vi "Read Sequence File.vi"(8 "error in":errorcluster, 11 "path":path) -> (0 "error out":errorcluster, 2 "rig config path":path, 3 "Sequence File":T1)   [LabVIEW 2026]
doc: "Reads a sequence JSON file as text and parses it with Parse Sequence JSON.vi into a Sequence File cluster; the rig config path is the sequence file folder joined with rig_config. An empty path returns error 7; a missing file, a JSON error or an empty steps array (error 5001) is passed out. AF-free."
uses:
  Typedefs/Condition.ctl
  Typedefs/Channel Value.ctl
  Typedefs/Step Config.ctl
  Typedefs/Sequence File.ctl
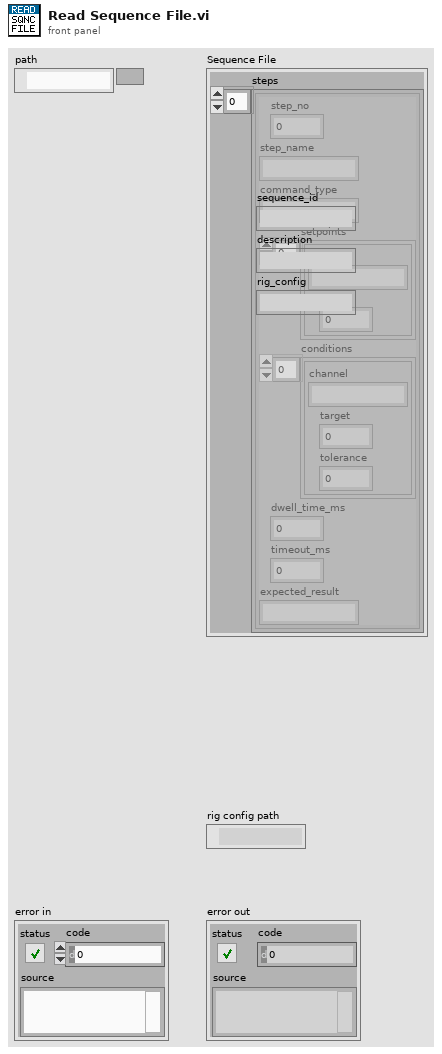
[diagram p1: front panel]
types:
  T1 = typedef "Sequence File.ctl" = cluster{"sequence_id":string, "description":string, "rig_config":string, "steps":T2[]}
  T2 = typedef "Step Config.ctl" = cluster{"step_no":i32, "step_name":string, "command_type":string, "setpoints":T3[], "conditions":T4[], "dwell_time_ms":i32, "timeout_ms":i32, "expected_result":string}
  T3 = typedef "Channel Value.ctl" = cluster{"channel":string, "value":dbl}
  T4 = typedef "Condition.ctl" = cluster{"channel":string, "target":dbl, "tolerance":dbl}
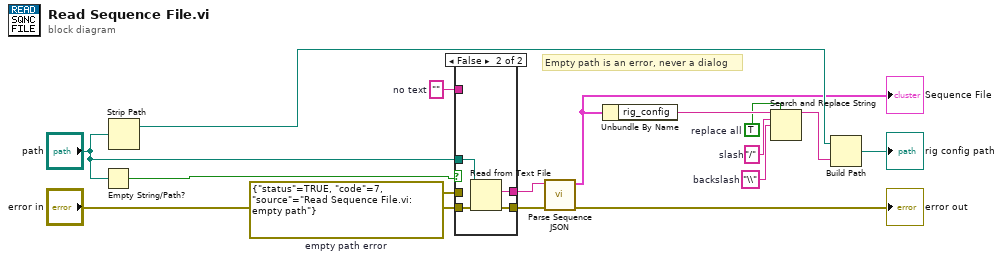
[diagram p0: block diagram]
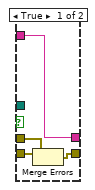
[diagram p2: hidden frame]
diagram:
  w6 = TRUE  # replace all
  w7 = "\\"  # backslash
  w8 = "/"  # slash
  w14 = ""  # no text
  w15 = errorcluster {"status"=TRUE, "code"=7, "source"="Read Sequence File.vi: empty path"}  # empty path error
  # "Empty path is an error, never a dialog"
  n1 = Empty String/Path?(string/path="path") -> (empty?=w13:bool)
  n2 = Strip Path(path="path") -> (stripped path=w5:path)  [unwired: 1 out]
  n3 = case shown="False" w13 {
    tunnel: "path" -> [_ w24]
    tunnel: "error in" -> [w20 w23]
    tunnel: w15 -> [w19 _]
    tunnel: [w18 w22] -> w12
    tunnel: w14 -> [w18 _]
    tunnel: [w17 w21] -> w11
    frame True {
      n4 = Merge Errors(w20, w19) -> (w17:errorcluster)
    }
    frame False {
      n5 = Read from Text File(file (use dialog)=w24, error in=w23) -> (text=w22:string, error out=w21:errorcluster)  [unwired: 2 in, 2 out]
    }
  }
  n6 = call "Parse Sequence JSON.vi"("error in"=w11, "JSON string"=w12) -> ("error out"=→"error out":errorcluster, "Sequence File"=w3:T1)  [unwired: 8 in]
  "Sequence File" <- w3
  n7 = Unbundle By Name(w3) -> ("rig_config"=w9:string)
  n8 = Search and Replace String(replace all?=w6, input string=w9, search string=w8, replace string=w7) -> (result string=w4:string)  [unwired: 4 in, 3 out]
  n9 = Build Path(base path=w5, name or relative path=w4) -> (appended path=→"rig config path":path)
